vi "T2.vi"() -> ()   [LabVIEW 2024]
uses:
  Global_Stop.vi
panel:
  in  "Use  Gate Commands?":bool
  in  "T set":string="5E3"
  in  "B Gate Delay":dbl=0.0004112
  in  "A Gate Delay":dbl=0.0002033
  out "At pass":i32
  in  "stop":bool
  in  "Number of individual passes?":i32
  in  "N":dbl=1.0
  out "DATA":dbl[][](array[numeric])
  in  "file path (use dialog) 3":path=path "C:/Users/Crawford Group/Desktop/Angelo/NMR/DATA/T2/Averaged.txt"
  in  "file path (use dialog) 2":path=path "C:/Users/Crawford Group/Desktop/Angelo/NMR/DATA/T2/B Gate.txt"
  in  "file path (use dialog)":path=path "C:/Users/Crawford Group/Desktop/Angelo/NMR/DATA/T2/A Gate.txt"
  out "A Gate":dbl[][](array[numeric])
  out "B Gate":dbl[][](array[numeric])
  out "data":dbl[](array[numeric])
  out "At step":i32
  out "Current Tau":dbl
  out "XY Graph":cluster{"Y":dbl[], "Y":dbl[]}[](graph)
  in  "Tau Step Size":dbl=2e-09
  in  "Number of steps":i32=500
  in  "Frequency in MHz":string="f2585"
  # "A gate Delay typically 20.82us\nB Gate delay typlically at 46.28 us"
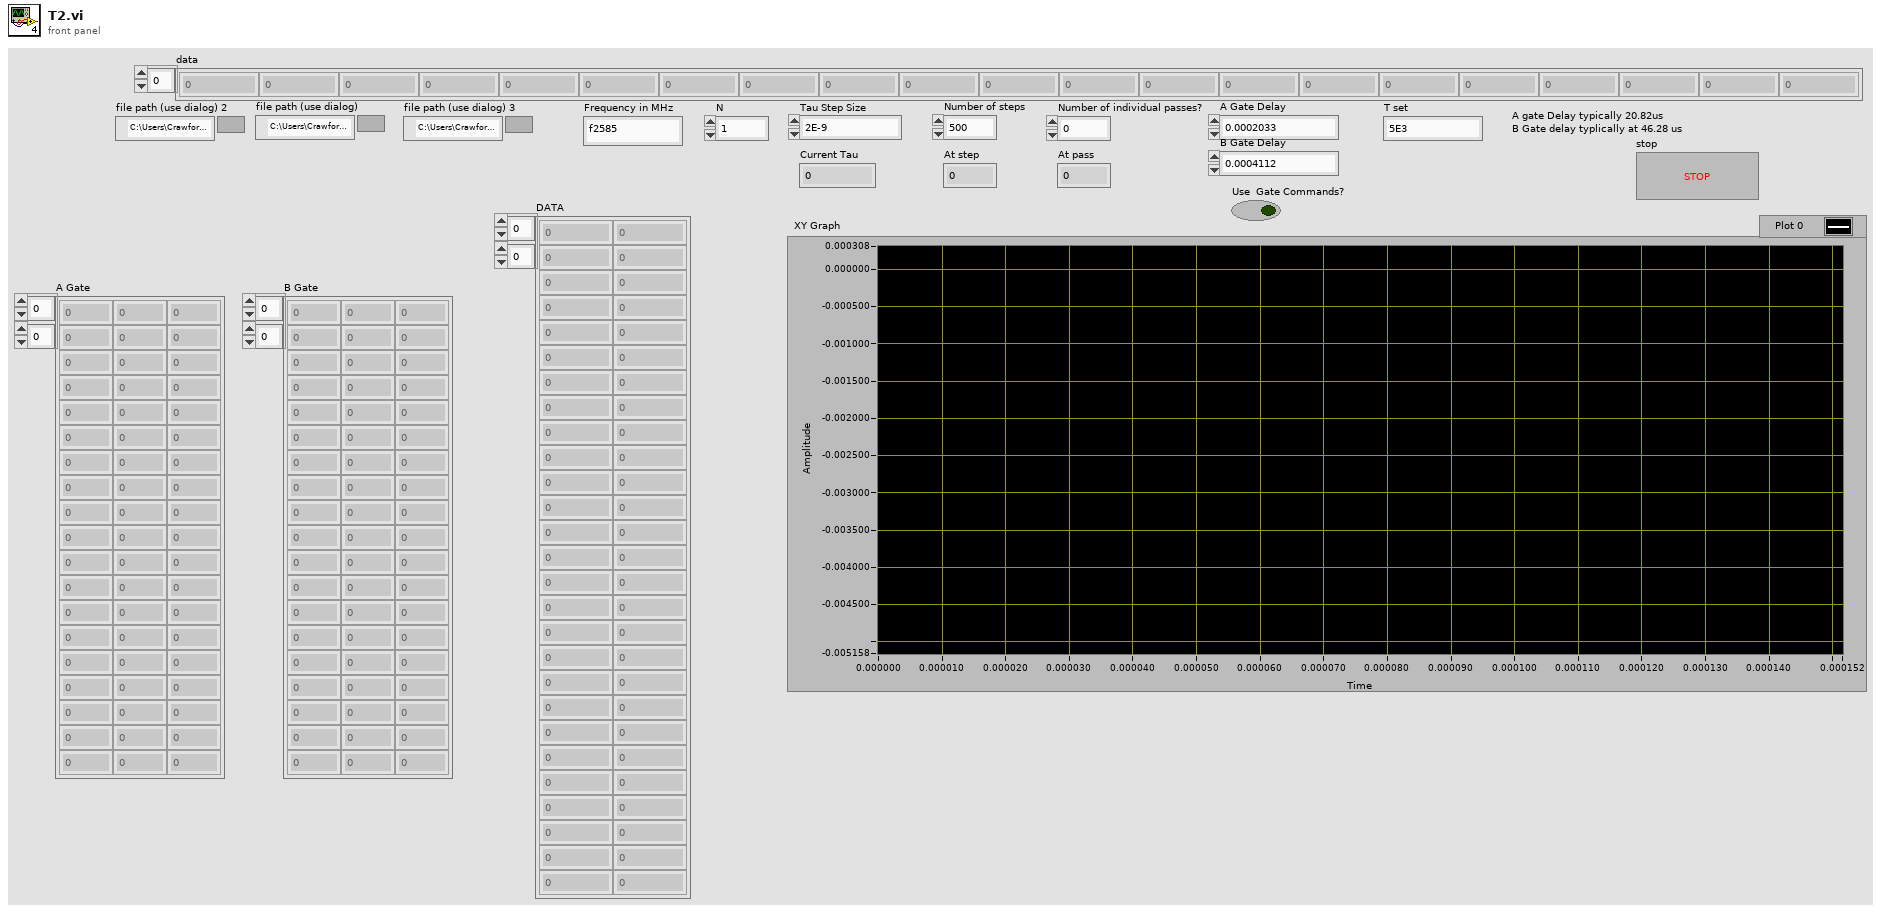
[diagram p1: front panel]
types:
  T1 = enum16{"open", "replace", "create", "open or create", "replace or create", "replace or create with confirmation"}
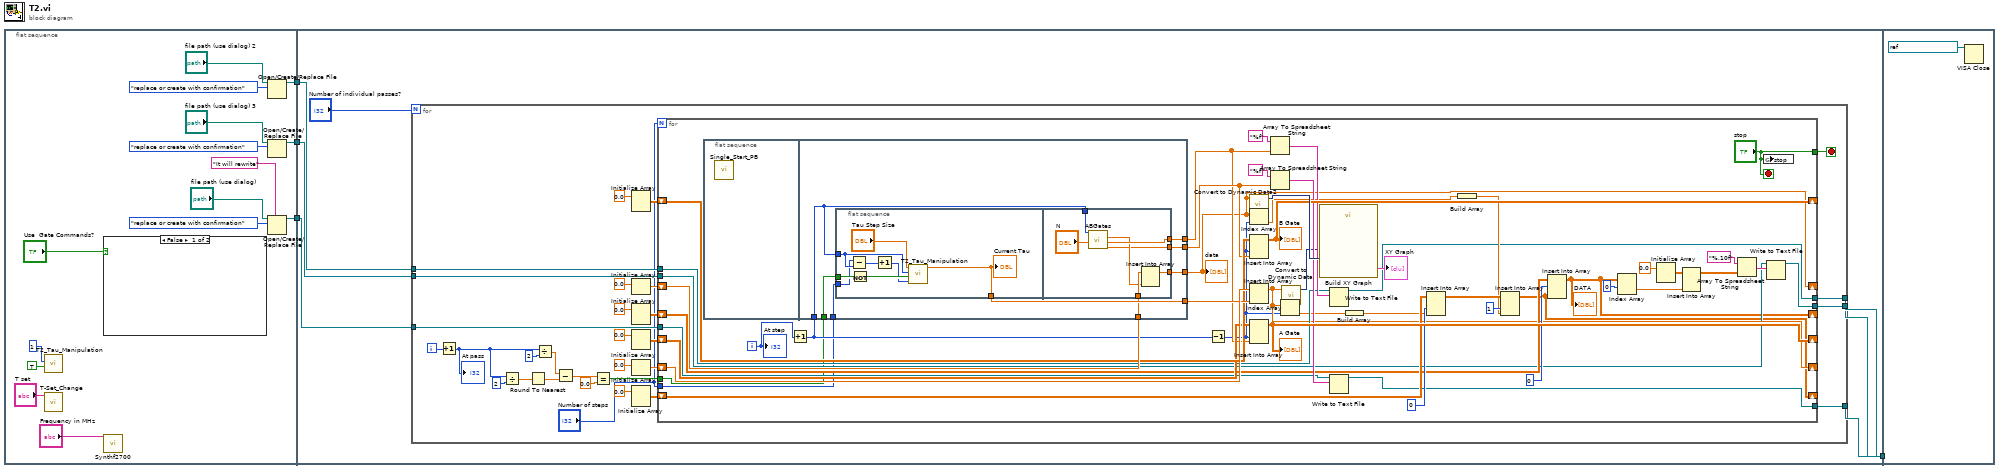
[diagram p0: block diagram]
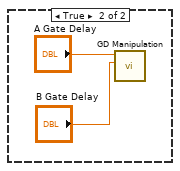
[diagram p2: hidden frame]
diagram:
  n1 = flat-sequence {
    tunnel: [w16] -> w6
    tunnel: [w13] -> w5
    tunnel: [w10] -> w4
    tunnel: w6 -> [w30]
    tunnel: w5 -> [w29]
    tunnel: w4 -> [w28]
    tunnel: [w27] -> w3
    tunnel: [w26] -> w2
    tunnel: [w25] -> w1
    tunnel: w3 -> [_]
    tunnel: w2 -> [_]
    tunnel: w1 -> [_]
    frame #0 {
      n2 = call "T2_Tau_Manipulation.vi"("Invert?"=TRUE, "Numeric"=1) -> ()  [unwired: 9 in, 1 out]
      n3 = call "T-Set_Change.vi"("T set"="T set") -> ()  [unwired: 11 in]
      n4 = case shown="False" "Use  Gate Commands?" {
        frame False {
        }
        frame True {
          n5 = call "GD Manipulation.vi"("B Gate delay"="B Gate Delay", "A Gate Delay"="A Gate Delay") -> ()  [unwired: 10 in]
        }
      }
      n6 = call "Synthf2700.vi"("Frequency in MHz"="Frequency in MHz") -> ()  [unwired: 11 in]
      n7 = Open/Create/Replace File(file path (use dialog)="file path (use dialog) 2", operation (0:open)=T1."replace or create with confirmation") -> (refnum out=w13:refnum<file>)  [unwired: 4 in, 2 out]
      n8 = Open/Create/Replace File(file path (use dialog)="file path (use dialog) 3", operation (0:open)=T1."replace or create with confirmation") -> (refnum out=w10:refnum<file>)  [unwired: 4 in, 2 out]
      n9 = Open/Create/Replace File(file path (use dialog)="file path (use dialog)", prompt="It will rewrite", operation (0:open)=T1."replace or create with confirmation") -> (refnum out=w16:refnum<file>)  [unwired: 3 in, 2 out]
    }
    frame #1 {
      n10 = for {
        N: "Number of individual passes?" -> [_]
        tunnel: w30 -> [w52]
        tunnel: [w45] -> w27
        tunnel: w28 -> [w46]
        tunnel: [w44] -> w26
        tunnel: w29 -> [w51]
        tunnel: [w43] -> w25
        i -> [w39]
        stop <- w31 stop-if-true
        n11 = Increment(x=w39) -> (x+1=w38:i32)
        "At pass" <- w38
        n12 = Divide(x=w38, y=2) -> (x/y=w35:dbl)
        n13 = Round To Nearest(number=w35) -> (nearest integer value=w34:dbl)
        n14 = Divide(x=w38, y=2) -> (x/y=w40:dbl)
        n15 = Subtract(x=w40, y=w34) -> (x-y=w37:dbl)
        n16 = Equal?(x=w37, y=0.0) -> (x = y?=w33:bool)
        n17 = Initialize Array(0.0) -> (w54:dbl[][])  [unwired: 2 in]
        n18 = Initialize Array(0.0) -> (w60:dbl[])  [unwired: 1 in]
        n19 = Initialize Array(0.0) -> (w47:dbl[][])  [unwired: 2 in]
        n20 = Initialize Array(0.0) -> (w53:dbl[][])  [unwired: 2 in]
        n21 = Initialize Array(0.0) -> (w59:dbl[])  [unwired: 1 in]
        n22 = Initialize Array(0.0) -> (w49:dbl[][])  [unwired: 2 in]
        n23 = for {
          N: "Number of steps" -> [_]
          shift-right: [w80] -> _
          shift-left: w60 -> [w109]
          shift-right: [w85] -> _
          shift-left: w59 -> [w108]
          shift-right: [w102] -> _
          shift-left: w54 -> [w105]
          shift-right: [w103] -> _
          shift-left: w53 -> [w104]
          tunnel: w52 -> [w100]
          tunnel: w51 -> [w96]
          shift-right: [w72] -> _
          shift-left: w49 -> [w90]
          shift-right: [w68] -> _
          shift-left: w47 -> [w89]
          tunnel: w46 -> [w76]
          tunnel: [w67] -> w45
          tunnel: [w66] -> w44
          tunnel: [w65] -> w43
          tunnel: w33 -> [w63]
          tunnel: "Number of steps" -> [w62]
          tunnel: ["stop"] -> w31
          i -> [w64]
          stop <- "stop" stop-if-true
          n24 = flat-sequence {
            tunnel: w86 -> [w112]
            tunnel: w109 -> [w114]
            tunnel: [w113] -> w80
            tunnel: [w117] -> w107
            tunnel: [w111] -> w95
            tunnel: [w110] -> w98
            tunnel: w63 -> [w116]
            tunnel: w62 -> [w115]
            frame #0 {
              n25 = call "Single_Start_PB.vi"() -> ()  [unwired: 12 in]
            }
            frame #1 {
              n26 = flat-sequence {
                tunnel: w112 -> [w125]
                tunnel: [w124] -> w117
                tunnel: w116 -> [w123]
                tunnel: w115 -> [w122]
                tunnel: w114 -> [w132]
                tunnel: [w131] -> w113
                tunnel: w112 -> [w130]
                tunnel: [w128] -> w111
                tunnel: [w126] -> w110
                frame #0 {
                  n27 = Subtract(x=w122, y=w125) -> (x-y=w119:i32)
                  n28 = Not(x=w123) -> (.not. x?=w121:bool)
                  n29 = Increment(x=w119) -> (x+1=w118:i32)
                  n30 = call "T2_Tau_Manipulation.vi"("Numeric 2"=w118, "Invert?"=w121, "Numeric"=w125, "MW Step Size"="Tau Step Size") -> ("Tau"=w124:dbl)  [unwired: 7 in]
                  "Current Tau" <- w124
                }
                frame #1 {
                  n31 = call "ABGates.vi"("N"="N", "# of loop"=w130) -> ("B Gate"=w126:dbl[], "A Gate"=w128:dbl[], "average A-B/A+B"=w127:dbl)  [unwired: 7 in]
                  n32 = Insert Into Array(array=w132, new element=w127) -> (w131:dbl[])  [unwired: 1 in]
                }
              }
            }
          }
          n33 = Increment(x=w64) -> (x+1=w86:i32)
          n34 = Decrement(x=w86) -> (x-1=w79:i32)
          n35 = call "Convert to Dynamic Data2"("Array"=w80) -> ("Dynamic Data Type"=w106:dynamicdata)  [unwired: 3 in]
          n36 = Index Array(array=w80, index=w79) -> (element=w82:dbl)
          n37 = Insert Into Array(array=w105, index (col)=w79, new element=w98) -> (w102:dbl[][])  [unwired: 1 in]
          "B Gate" <- w102
          n38 = Insert Into Array(array=w108, new element=w107) -> (w85:dbl[])  [unwired: 1 in]
          n39 = Insert Into Array(array=w104, index (col)=w79, new element=w95) -> (w103:dbl[][])  [unwired: 1 in]
          "A Gate" <- w103
          n40 = Array To Spreadsheet String(array=w95, 3:"%f" ("format string")) -> (spreadsheet string=w97:string)  [unwired: 1 in]
          n41 = Array To Spreadsheet String(array=w98, 3:"%f" ("format string")) -> (spreadsheet string=w101:string)  [unwired: 1 in]
          n42 = Index Array(array=w85, index=w79) -> (element=w84:dbl)
          n43 = call "Convert to Dynamic Data"("Array"=w85) -> ("Dynamic Data Type"=w87:dynamicdata)  [unwired: 3 in]
          n44 = call "Build XY Graph"("Y Input"=w106, "X Input"=w87) -> ("XY Graph"=→"XY Graph":cluster{"X":dbl[], "Y":dbl[]}[])  [unwired: 8 in, 1 out]
          n45 = Write to Text File(file (use dialog)=w96, text=w97) -> (refnum out=w66:refnum<file>)  [unwired: 2 in, 2 out]
          n46 = Write to Text File(file (use dialog)=w100, text=w101) -> (refnum out=w67:refnum<file>)  [unwired: 2 in, 2 out]
          n47 = Build Array(w84) -> (w83:dbl[])
          n48 = Insert Into Array "Insert Into Array"(array=w90, index (col)=0 ("disabled index (col)"), new element=w83) -> (w91:dbl[][])  [unwired: 1 in]
          n49 = Build Array(w82) -> (w81:dbl[])
          n50 = Insert Into Array(array=w91, index (col)=1 ("disabled index (col)"), new element=w81) -> (w72:dbl[][])  [unwired: 1 in]
          n51 = Insert Into Array(array=w89, index (row)=0, new element=w72) -> (w68:dbl[][])  [unwired: 1 in]
          "DATA" <- w68
          n52 = Index Array(array=w68, index (row)=0) -> (element=w70:dbl[])  [unwired: 1 in]
          n53 = Initialize Array(0.0 ("element")) -> (w69:dbl[][])  [unwired: 2 in]
          n54 = Insert Into Array(array=w69, new element=w70) -> (w73:dbl[][])  [unwired: 2 in]
          n55 = Array To Spreadsheet String(array=w73, 3:"%.10f" ("format string")) -> (spreadsheet string=w77:string)  [unwired: 1 in]
          n56 = global write "Global_Stop.vi" "stop"("stop") -> ()
          n57 = Write to Text File(file (use dialog)=w76, text=w77) -> (refnum out=w65:refnum<file>)  [unwired: 2 in, 2 out]
          "At step" <- w64
          "data" <- w80
        }
      }
    }
    frame #2 {
      n58 = VISA Close(VISA resource name=refnum<visa-resource-name> "GPIB0::23::INSTR") -> ()  [unwired: 1 in, 1 out]
    }
  }
